vi "Send Default Response.vi"(8 "error in (no error)":errorcluster caption="에러 입력(에러 없음)", 10 "id":string, 11 "Instrument Manager 입력":refnum<class "Instrument Manager.lvclass">) -> (0 "error out":errorcluster caption="에러 출력", 3 "Instrument Manager 출력":refnum<class "Instrument Manager.lvclass">)   [LabVIEW 2023, in "Instrument Manager.lvclass"]
uses:
  Instrument Manager.lvclass
  Default Response.ctl
  Instrument Manager.lvclass/Instrument Manager.ctl
  Error Response.ctl
panel:
  out "JSON 문자열":string
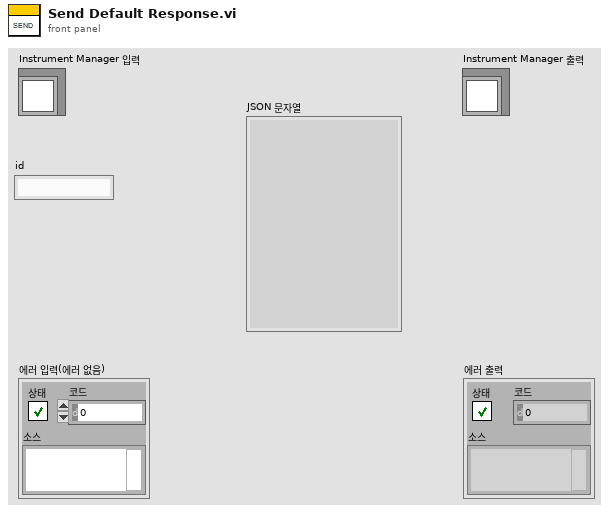
[diagram p1: front panel]
types:
  T1 = typedef "Instrument Manager.lvclass/Default Response.ctl" = cluster{"type":string, "id":string, "status":string}
  T2 = cluster{"Reader Q":refnum<queue>, "Writer Q":refnum<queue>}
  T3 = typedef "Instrument Manager.lvclass/Error Response.ctl" = cluster{"type":string, "id":string, "status":string, "error out":errorcluster}
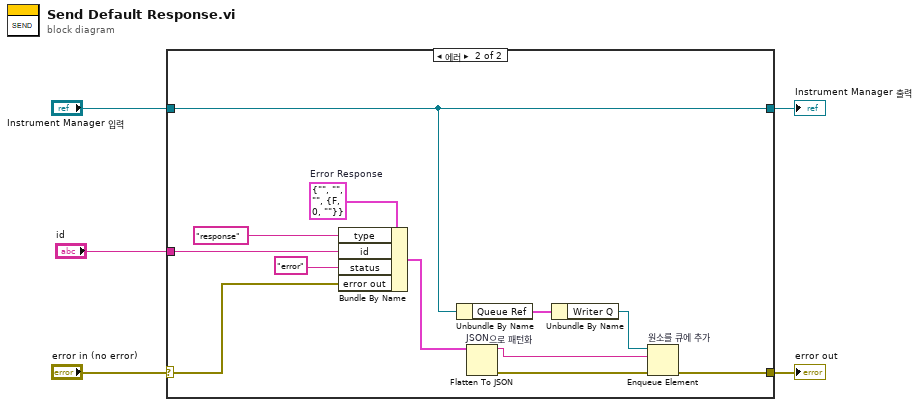
[diagram p0: block diagram]
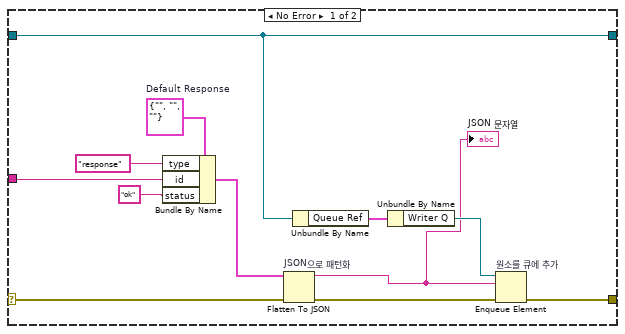
[diagram p2: hidden frame]
diagram:
  n1 = case shown="에러" "error in (no error)" {
    selector: "error in (no error)" -> [w15 w28]
    tunnel: [w12 w19] -> w4
    tunnel: [w17 w24] -> w2
    tunnel: "Instrument Manager 입력" -> [w17 w24]
    tunnel: "id" -> [w9 w18]
    frame No Error {
      w11 = T1 {"type"="", "id"="", "status"=""}  # Default Response
      n2 = Bundle By Name(cluster=w11, "type"="response", "id"=w9, "status"="ok") -> (w10:T1)
      n3 = Flatten To JSON "JSON으로 패턴화"(anything=w10, error in (no error)=w15) -> (JSON string=w6:string, 11:w14:errorcluster)  [unwired: 1 in]
      "JSON 문자열" <- w6
      n4 = Unbundle By Name(w17) -> ("Queue Ref"=w16:T2)
      n5 = Unbundle By Name(w16) -> ("Writer Q"=w13:refnum<queue>)
      n6 = Enqueue Element "원소를 큐에 추가"(queue=w13, element=w6, error in (no error)=w14) -> (error out=w12:errorcluster)  [unwired: 1 in, 2 out]
    }
    frame Error {
      w29 = T3 {"type"="", "id"="", "status"="", "error out"={"status"=FALSE, "code"=0, "source"=""}}  # Error Response
      n7 = Bundle By Name(cluster=w29, "type"="response", "id"=w18, "status"="error", "error out"=w28) -> (w21:T3)
      n8 = Unbundle By Name(w24) -> ("Queue Ref"=w27:T2)
      n9 = Flatten To JSON "JSON으로 패턴화"(anything=w21) -> (JSON string=w25:string, 11:w20:errorcluster)  [unwired: 2 in]
      n10 = Unbundle By Name(w27) -> ("Writer Q"=w26:refnum<queue>)
      n11 = Enqueue Element "원소를 큐에 추가"(queue=w26, element=w25, error in (no error)=w20) -> (error out=w19:errorcluster)  [unwired: 1 in, 2 out]
    }
  }
  "error out" <- w4
  "Instrument Manager 출력" <- w2
